vi "Runtime_Initialize.vi"(8 "error in (no error)":errorcluster={"status"=FALSE, "code"=0, "source"="\"\""}, 10 "configuration locations":string, 11 "Target capability":string) -> (0 "error out":errorcluster={"status"=FALSE, "code"=0, "source"="\"\""}, 2 "status ok":bool, 3 "Service references":string)   [LabVIEW 2026]
doc: "INTENT: Prepare registries/queues/loggers. LOGIC: Create bounded message queues, event log, registry, Bridge, RT gateway and simulator selection."
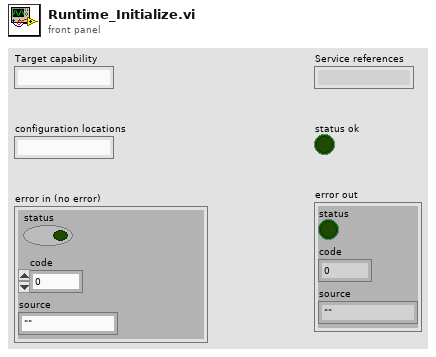
[diagram p1: front panel]
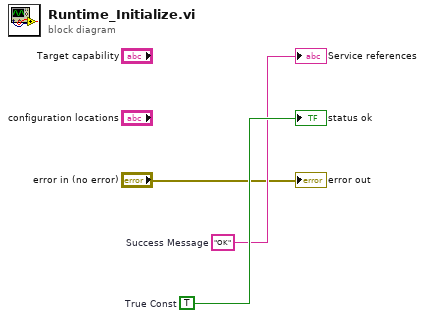
[diagram p0: block diagram]
diagram:
  w3 = TRUE  # True Const
  w2 = "OK"  # Success Message
  "Service references" <- w2
  "status ok" <- w3
  "error out" <- "error in (no error)"
